vi "Main On Load Action VI.vi"(8 "error in (no error)":errorcluster, 11 "Device Item Ref in":T1 format="%.0x") -> (0 "error out":errorcluster, 3 "Device Item Ref out":T1 format="%.0x")   [LabVIEW 2015, in "Engine Simulation Toolkit System Explorer.lvlib"]
uses:
  Engine Simulation Toolkit System Explorer.lvlib
  <vilib>/NI Veristand/Custom Device API/Custom Device Item Ref.ctl
  NationalInstruments.VeriStand.SystemDefinitionAPI
  Shared/Constants and GUIDs.vi
  Shared/Properties.vi
  <vilib>/NI Veristand/Custom Device API/Get Item Property (String).vi
  <vilib>/NI Veristand/Custom Device API/Set Item Property (String).vi
  <vilib>/NI Veristand/Custom Device API/Get Item Property (Dependent File).vi
  <vilib>/NI Veristand/Custom Device API/Set Item Property (Dependent File).vi
  <vilib>/NI Veristand/Custom Device Tools/Custom Device Utility Library/NI VeriStand - Search for All Items by GUID.vi
  <vilib>/NI Veristand/Custom Device Tools/Custom Device Utility Library/NI VeriStand - Search for Item by Name.vi
  <vilib>/NI Veristand/Custom Device API/Custom Device API.lvlib
  Shared/Engine Simulation Toolkit Shared.lvlib
  <vilib>/NI Veristand/Custom Device Tools/Custom Device Utility Library/Custom Device Utility Library.lvlib
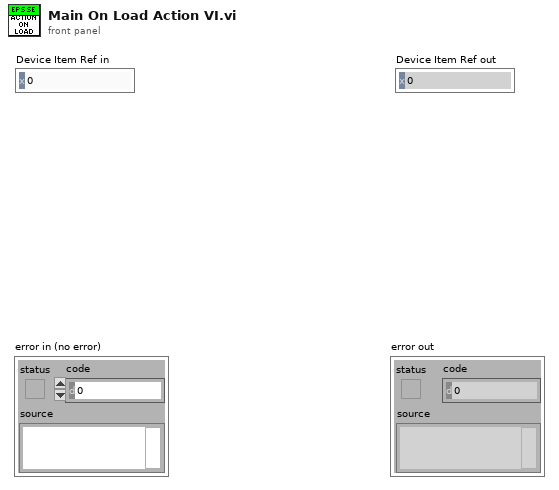
[diagram p1: front panel]
types:
  T1 = typedef "Custom Device API.lvlib/Custom Device Item Ref.ctl" = u64
  T2 = typedef "Custom Device API.lvlib/Dependent File Optional Info.ctl" = cluster{"Version":string, "RTDestination":path, "ForceDownload":bool, "SupportedTarget":string, "MD5":string}
  T3 = typedef "Engine Simulation Toolkit Shared.lvlib/Channel.ctl" = cluster{"Name":string, "Units":string, "Default":dbl, "Description":string, "Scalable":bool}
  T4 = cluster{"GUID.APU Commands":string, "ChanList.APU Commands":T3[]}
  T5 = cluster{"GUID.APU State":string, "ChanList.APU State":T3[]}
  T6 = cluster{"GUID.Analog Replay":string, "ChanList.DataReplayVoltage":T3[]}
  T7 = cluster{"GUID.Faulting":string, "ChanList.DigPtrnFaultingIn":T3[]}
  T8 = cluster{"GUID.Faulting":string, "ChanList.DigPtrnFaultingOut":T3[]}
  T9 = cluster{"GUID.Dir Speed Sensor":string, "ChanList.DirSpeedSensor":T3[]}
  T10 = cluster{"GUID.Event Capture":string, "ChanList.EventCapture":T3[]}
  T11 = cluster{"GUID.Knock Cylinder":string, "ChanList.KnockCylinder":T3[]}
  T12 = cluster{"GUID.Knock Sensor":string, "ChanList.KnockSensor":T3[]}
  T13 = cluster{"GUID.APU State":string, "ChanList.MeasurementStatus":T3[]}
  T14 = cluster{"GUID.Analog Replay":string, "ChanList.Offset":T3[]}
  T15 = cluster{"GUID.Digital Pattern":string, "ChanList.Offset":T3[]}
  T16 = cluster{"GUID.Status":string, "ChanList.Status Chans":T3[]}
  T17 = cluster{"GUID.Status":string, "ChanList.Status Chans":T3[]}[]
  T18 = typedef "Custom Device API.lvlib/Custom Device Item Info.ctl" = cluster{"Name":string, "Is Channel":bool, "GUID":string, "Is Waveform":bool}
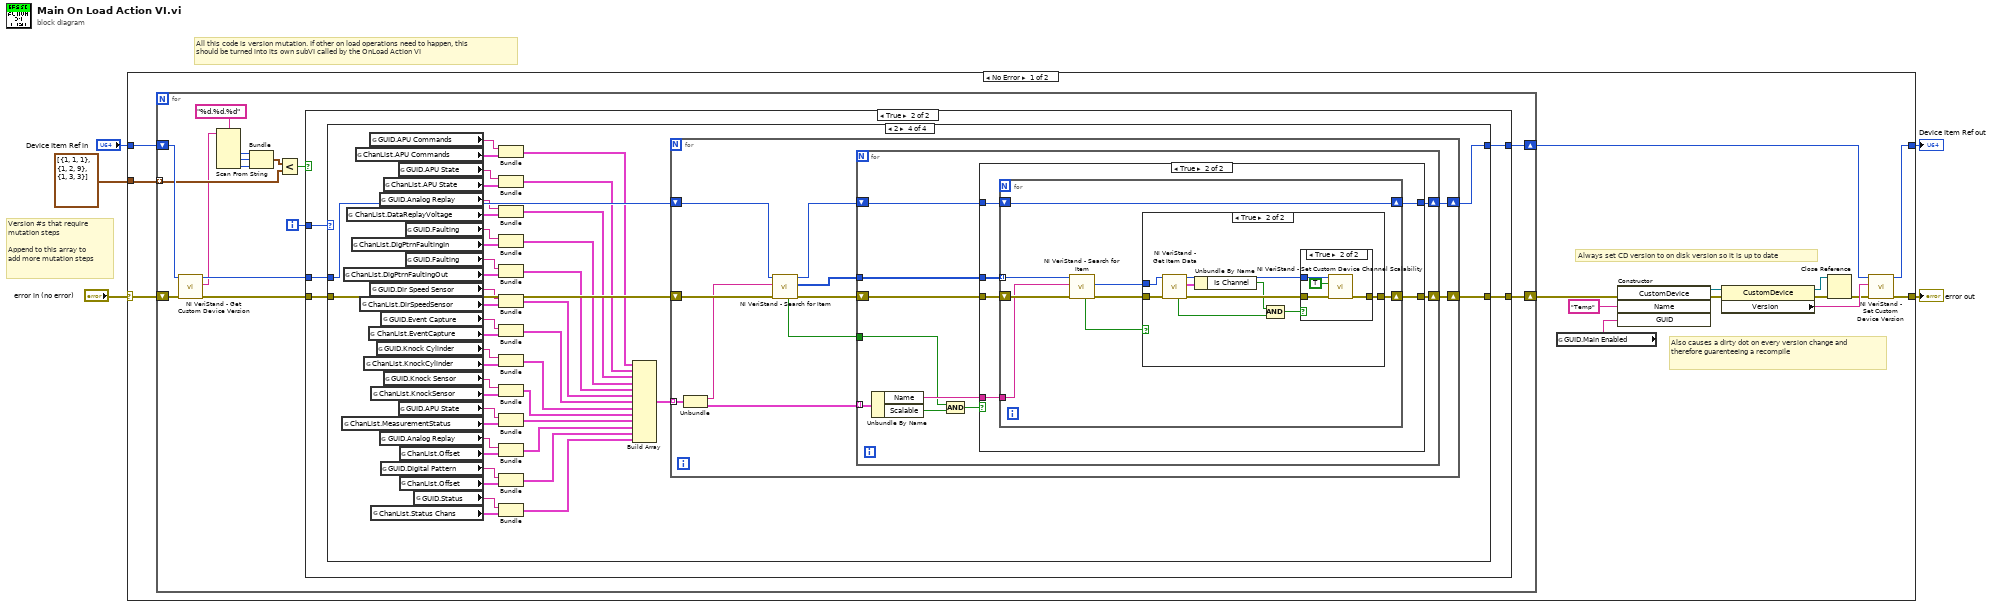
[diagram p0: block diagram]
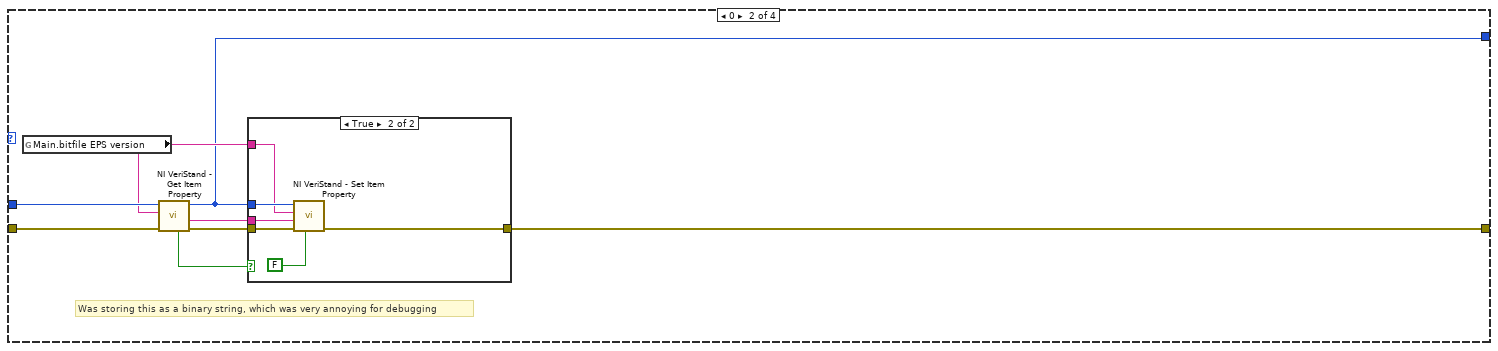
[diagram p4: hidden frame]
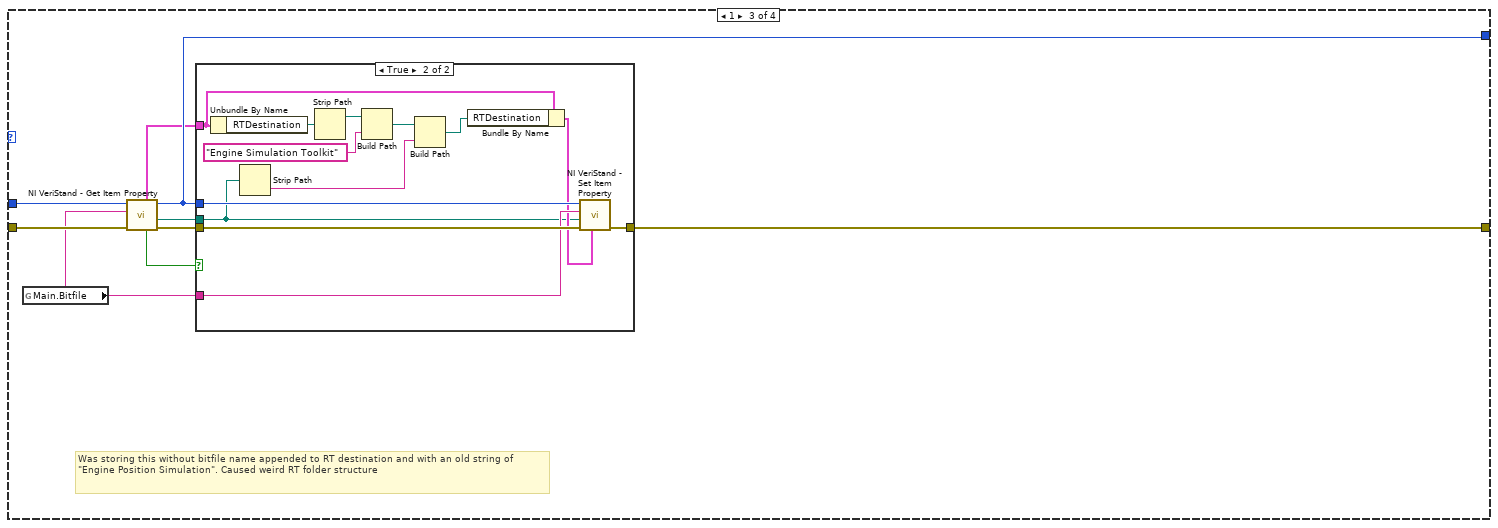
[diagram p6: hidden frame]
diagram:
  # "All this code is version mutation. If other on load operations need to happen, this should be turned into its own subVI called by the OnLoad Action VI"
  # "Version #s that require\nmutation steps\n\nAppend to this array to\nadd more mutation steps"
  n1 = case shown="No Error" "error in (no error)" {
    selector: "error in (no error)" -> [w19 w180]
    tunnel: [w9 w180] -> w4
    tunnel: "Device Item Ref in" -> [w18 w179]
    tunnel: [w7 w179] -> w2
    tunnel: cluster{i32, i32, i32}[] [{1, 1, 1}, {1, 2, 9}, {1, 3, 3}] -> [w20 _]
    frame No Error {
      # "Also causes a dirty dot on every version change and therefore guarenteeing a recompile"
      # "Always set CD version to on disk version so it is up to date"
      n2 = for {
        tunnel: w20 -> [w23] mode=indexing
        shift-right: [w27] -> w10
        shift-left: w19 -> [w31]
        shift-right: [w25] -> w8
        shift-left: w18 -> [w30]
        i -> [w24]
        n3 = call <vilib>:"NI VeriStand - Get Custom Device Version.vi"("error in (no error)"=w31, "Device Ref in"=w30) -> ("error out"=w28:errorcluster, "Value"=w21:string, "Device Ref out"=w26:T1)  [unwired: 7 in]
        n4 = Scan From String(format string="%d.%d.%d", input string=w21) -> (output 1=w33:i32, output 2=w34:i32, output 3=w22:i32)  [unwired: 5 in, 3 out]
        n5 = Bundle(w33, w34, w22) -> (w35:cluster{i32, i32, i32})  [unwired: 1 in]
        n6 = Less?(x=w35, y=w23) -> (x < y?=w29:bool)
        n7 = case shown="True" w29 {
          tunnel: w28 -> [w37 w42]
          tunnel: [w37 w41] -> w27
          tunnel: w26 -> [w36 w38]
          tunnel: [w36 w39] -> w25
          tunnel: w24 -> [_ w40]
          frame False {
          }
          frame True {
            n8 = case shown="2" w40 {
              tunnel: w42 -> [w44 w51 w67 w125]
              tunnel: [w44 w46 w62 w124] -> w41
              tunnel: [w43 w45 w61 w123] -> w39
              tunnel: w38 -> [w43 w52 w68 w126]
              frame Default {
              }
              frame 0 {
                # "Was storing this as a binary string, which was very annoying for debugging"
                n9 = global read "Properties.vi" "Main.bitfile EPS version"() -> (w48:string)
                n10 = call-poly <vilib>:"NI VeriStand - Get Item Property.vi"("error in (no error)"=w51, "Property Name"=w48, "Item Ref in"=w52) -> ("error out"=w49:errorcluster, "Value"=w47:string, "Item Ref out"=w45:T1, "Found?"=w50:bool)  [unwired: 5 in]
                n11 = case shown="True" w50 {
                  tunnel: w45 -> [_ w59]
                  tunnel: w49 -> [w53 w58]
                  tunnel: w48 -> [_ w57]
                  tunnel: w47 -> [_ w56]
                  tunnel: [w53 w54] -> w46
                  frame False {
                  }
                  frame True {
                    n12 = call-poly <vilib>:"NI VeriStand - Set Item Property.vi"("Binary String (T)"=FALSE, "error in (no error)"=w58, "Value"=w56, "Property Name"=w57, "Item Ref in"=w59) -> ("error out"=w54:errorcluster)  [unwired: 4 in, 2 out]
                  }
                }
              }
              frame 1 {
                # "Was storing this without bitfile name appended to RT destination and with an old string of \"Engine Position Simulation\". Caused weird RT folder structure"
                n13 = global read "Properties.vi" "Main.Bitfile"() -> (w64:string)
                n14 = call-poly <vilib>:"NI VeriStand - Get Item Property.vi"("error in (no error)"=w67, "Property Name"=w64, "Item Ref in"=w68) -> ("error out"=w65:errorcluster, "Path"=w63:path, "Item Ref out"=w61:T1, "Found"=w66:bool, "OptionalInfo"=w60:T2)  [unwired: 4 in]
                n15 = case shown="True" w66 {
                  tunnel: w61 -> [_ w82]
                  tunnel: w65 -> [w69 w81]
                  tunnel: w64 -> [_ w80]
                  tunnel: w63 -> [_ w75]
                  tunnel: [w69 w79] -> w62
                  tunnel: w60 -> [_ w78]
                  frame False {
                  }
                  frame True {
                    n16 = Unbundle By Name(w78) -> ("RTDestination"=w74:path)
                    n17 = Strip Path(path=w75) -> (name=w76:string)  [unwired: 1 out]
                    n18 = Strip Path(path=w74) -> (stripped path=w73:path)  [unwired: 1 out]
                    n19 = Build Path(base path=w73, name or relative path="Engine Simulation Toolkit") -> (appended path=w72:path)
                    n20 = Build Path(base path=w72, name or relative path=w76) -> (appended path=w70:path)
                    n21 = Bundle By Name(cluster=w78, "RTDestination"=w70) -> (w77:T2)
                    n22 = call-poly <vilib>:"NI VeriStand - Set Item Property.vi"("OptionalInfo"=w77, "error in (no error)"=w81, "Path"=w75, "Property Name"=w80, "Item Ref in"=w82) -> ("error out"=w79:errorcluster)  [unwired: 4 in, 2 out]
                  }
                }
              }
              frame 2 {
                n23 = global read "Constants and GUIDs.vi" "ChanList.MeasurementStatus"() -> (w102:T3[])
                n24 = global read "Constants and GUIDs.vi" "ChanList.DigPtrnFaultingOut"() -> (w112:T3[])
                n25 = global read "Constants and GUIDs.vi" "ChanList.DataReplayVoltage"() -> (w118:T3[])
                n26 = global read "Constants and GUIDs.vi" "ChanList.DigPtrnFaultingIn"() -> (w117:T3[])
                n27 = global read "Constants and GUIDs.vi" "ChanList.APU Commands"() -> (w121:T3[])
                n28 = global read "Constants and GUIDs.vi" "ChanList.DirSpeedSensor"() -> (w110:T3[])
                n29 = global read "Constants and GUIDs.vi" "ChanList.KnockCylinder"() -> (w106:T3[])
                n30 = global read "Constants and GUIDs.vi" "ChanList.EventCapture"() -> (w108:T3[])
                n31 = global read "Constants and GUIDs.vi" "GUID.APU Commands"() -> (w116:string)
                n32 = global read "Constants and GUIDs.vi" "GUID.Dir Speed Sensor"() -> (w109:string)
                n33 = global read "Constants and GUIDs.vi" "ChanList.KnockSensor"() -> (w104:T3[])
                n34 = global read "Constants and GUIDs.vi" "ChanList.Status Chans"() -> (w96:T3[])
                n35 = global read "Constants and GUIDs.vi" "GUID.Knock Cylinder"() -> (w105:string)
                n36 = global read "Constants and GUIDs.vi" "GUID.Analog Replay"() -> (w114:string)
                n37 = global read "Constants and GUIDs.vi" "GUID.Analog Replay"() -> (w99:string)
                n38 = global read "Constants and GUIDs.vi" "GUID.Digital Pattern"() -> (w97:string)
                n39 = global read "Constants and GUIDs.vi" "GUID.Event Capture"() -> (w107:string)
                n40 = global read "Constants and GUIDs.vi" "ChanList.APU State"() -> (w119:T3[])
                n41 = global read "Constants and GUIDs.vi" "GUID.Knock Sensor"() -> (w103:string)
                n42 = global read "Constants and GUIDs.vi" "GUID.APU State"() -> (w115:string)
                n43 = global read "Constants and GUIDs.vi" "GUID.APU State"() -> (w101:string)
                n44 = global read "Constants and GUIDs.vi" "ChanList.Offset"() -> (w100:T3[])
                n45 = global read "Constants and GUIDs.vi" "ChanList.Offset"() -> (w98:T3[])
                n46 = global read "Constants and GUIDs.vi" "GUID.Faulting"() -> (w113:string)
                n47 = global read "Constants and GUIDs.vi" "GUID.Faulting"() -> (w111:string)
                n48 = global read "Constants and GUIDs.vi" "GUID.Status"() -> (w95:string)
                n49 = Bundle("GUID.APU Commands"=w116, "ChanList.APU Commands"=w121) -> (w120:T4)  [unwired: 1 in]
                n50 = Bundle("GUID.APU State"=w115, "ChanList.APU State"=w119) -> (w94:T5)  [unwired: 1 in]
                n51 = Bundle("GUID.Analog Replay"=w114, "ChanList.DataReplayVoltage"=w118) -> (w93:T6)  [unwired: 1 in]
                n52 = Bundle("GUID.Faulting"=w113, "ChanList.DigPtrnFaultingIn"=w117) -> (w92:T7)  [unwired: 1 in]
                n53 = Bundle("GUID.Faulting"=w111, "ChanList.DigPtrnFaultingOut"=w112) -> (w91:T8)  [unwired: 1 in]
                n54 = Bundle("GUID.Dir Speed Sensor"=w109, "ChanList.DirSpeedSensor"=w110) -> (w90:T9)  [unwired: 1 in]
                n55 = Bundle("GUID.Event Capture"=w107, "ChanList.EventCapture"=w108) -> (w89:T10)  [unwired: 1 in]
                n56 = Bundle("GUID.Knock Cylinder"=w105, "ChanList.KnockCylinder"=w106) -> (w88:T11)  [unwired: 1 in]
                n57 = Bundle("GUID.Knock Sensor"=w103, "ChanList.KnockSensor"=w104) -> (w87:T12)  [unwired: 1 in]
                n58 = Bundle("GUID.APU State"=w101, "ChanList.MeasurementStatus"=w102) -> (w86:T13)  [unwired: 1 in]
                n59 = Bundle("GUID.Analog Replay"=w99, "ChanList.Offset"=w100) -> (w85:T14)  [unwired: 1 in]
                n60 = Bundle("GUID.Digital Pattern"=w97, "ChanList.Offset"=w98) -> (w84:T15)  [unwired: 1 in]
                n61 = Bundle("GUID.Status"=w95, "ChanList.Status Chans"=w96) -> (w83:T16)  [unwired: 1 in]
                n62 = Build Array(w120, w94, w93, w92, w91, w90, w89, w88, w87, w86, w85, w84, w83) -> (w122:T17)
                n63 = for {
                  shift-right: [w136] -> w123
                  shift-left: w126 -> [w137]
                  shift-right: [w134] -> w124
                  shift-left: w125 -> [w135]
                  tunnel: w122 -> [w129] mode=indexing
                  n64 = Unbundle(w129) -> ("GUID.Status"=w127:string, "ChanList.Status Chans"=w128:T3[])
                  n65 = call-poly <vilib>:"NI VeriStand - Search for Item.vi"("error in"=w135, "Item GUID"=w127, "Section Ref in"=w137) -> ("error out"=w130:errorcluster, "Item Refs"=w133:T1[], "Section Ref out"=w131:T1, "Found"=w132:bool)  [unwired: 5 in]
                  n66 = for {
                    tunnel: w128 -> [w145] mode=indexing
                    tunnel: w133 -> [w143]
                    tunnel: w132 -> [w139]
                    shift-right: [w147] -> w136
                    shift-left: w131 -> [w142]
                    shift-right: [w146] -> w134
                    shift-left: w130 -> [w141]
                    n67 = Unbundle By Name(w145) -> ("Name"=w144:string, "Scalable"=w140:bool)
                    n68 = Compound Arithmetic op=AND(w139, w140) -> (w138:bool)
                    n69 = case shown="True" w138 {
                      tunnel: [w149 w150] -> w147
                      tunnel: w141 -> [w148 w155]
                      tunnel: [w148 w154] -> w146
                      tunnel: w144 -> [_ w153]
                      tunnel: w143 -> [_ w152]
                      tunnel: w142 -> [w149 w151]
                      frame False {
                      }
                      frame True {
                        n70 = for {
                          tunnel: w153 -> [w159]
                          tunnel: w152 -> [w157] mode=indexing
                          shift-right: [w160] -> w154
                          shift-left: w155 -> [w161]
                          shift-right: [w156] -> w150
                          shift-left: w151 -> [w156]
                          n71 = call-poly <vilib>:"NI VeriStand - Search for Item.vi"("error in"=w161, "Item Name"=w159, "Section Ref in"=w157) -> ("error out"=w163:errorcluster, "Item Ref"=w162:T1, "Found"=w158:bool)  [unwired: 5 in, 1 out]
                          n72 = case shown="True" w158 {
                            tunnel: w163 -> [w164 w173]
                            tunnel: w162 -> [_ w172]
                            tunnel: [w164 w171] -> w160
                            frame False {
                            }
                            frame True {
                              n73 = call <vilib>:"NI VeriStand - Get Item Data.vi"("error in (no error)"=w173, "Item Ref in"=w172) -> ("error out"=w168:errorcluster, "Item Info"=w170:T18, "Item Ref out"=w169:T1, "Found"=w167:bool)  [unwired: 6 in]
                              n74 = Unbundle By Name(w170) -> ("Is Channel"=w166:bool)
                              n75 = Compound Arithmetic op=AND(w166, w167) -> (w165:bool)
                              n76 = case shown="True" w165 {
                                tunnel: w169 -> [_ w178]
                                tunnel: w168 -> [w174 w177]
                                tunnel: [w174 w176] -> w171
                                frame False {
                                }
                                frame True {
                                n77 = call <vilib>:"NI VeriStand - Set Custom Device Channel Scalability.vi"("error in (no error)"=w177, "Scalability"=TRUE, "Channel Ref in"=w178) -> ("error out"=w176:errorcluster)  [unwired: 7 in, 1 out]
                                }
                              }
                            }
                          }
                        }
                      }
                    }
                  }
                }
              }
            }
          }
        }
      }
      n78 = global read "Constants and GUIDs.vi" "GUID.Main Enabled"() -> (w6:string)
      n79 = constructor class="CustomDevice"(error in=w10, "Name"="Temp", "GUID"=w6) -> (reference out=w16:refnum<k24>, error out=w15:errorcluster)  [unwired: 2 in, 3 out]
      n80 = property class="CustomDevice"(reference=w16, error in=w15) -> (reference out=w13:refnum<k24>, error out=w14:errorcluster, "Version"=w12:string)
      n81 = Close Reference(reference=w13, error in (no error)=w14) -> (error out=w11:errorcluster)
      n82 = call <vilib>:"NI VeriStand - Set Custom Device Version.vi"("error in (no error)"=w11, "Value"=w12, "Device Ref in"=w8) -> ("error out"=w9:errorcluster, "Device Ref out"=w7:T1)  [unwired: 7 in]
    }
    frame Error {
    }
  }
  "error out" <- w4
  "Device Item Ref out" <- w2
